vi "GDSLvIcon_GenerateIconText.vi"(1 "Text":T2, 2 "TextPixelHeight(5-30)":i32=7, 3 "Foreground color":u32(colorbox), 4 "Background color":u32(colorbox)=16777215, 5 "error in (no error)":errorcluster, 6 "Offset":cluster{"X":i32, "Y":i32}, 7 "Text Pixel width(32-FrameThicknes*2))":i32=30) -> (14 "X-Limited":bool, 15 "Y-Limited":bool, 17 "TextOut":u8[][](array[numeric]), 18 "TextBounds":T1, 19 "error out":errorcluster)   [LabVIEW 2020]
doc: "Applies a text in the template picture."
uses:
  <resource>/Framework/Providers/Open_GDS/ClassProviders/Common/LvIcon_class/subvis/GDSLvIcon_TextDataType.ctl
  <resource>/Framework/Providers/Open_GDS/ClassProviders/Common/LvIcon_class/GDSLvIcon_WordCompressionType.ctl
  <resource>/Framework/Providers/Open_GDS/ClassProviders/Common/LvIcon_class/GDSLvIcon_TextAlignment.ctl
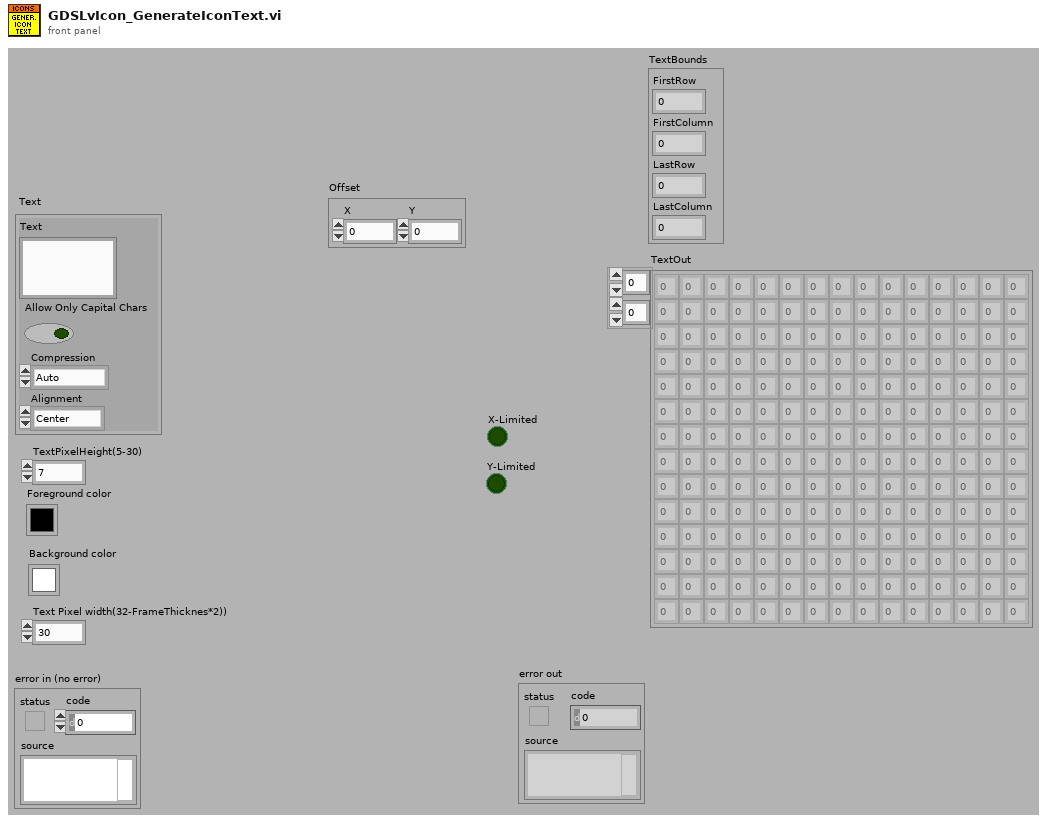
[diagram p1: front panel]
types:
  T1 = cluster{"FirstRow":i32, "FirstColumn":i32, "LastRow":i32, "LastColumn":i32}
  T2 = typedef "GDSLvIcon_TextDataType.ctl" = cluster{"Text":string, "Allow Only Capital Chars":bool, "Compression":T3, "Alignment":T4}
  T3 = typedef "GDSLvIcon_WordCompressionType.ctl" = enum16{"Auto", "On", "Off"}
  T4 = typedef "GDSLvIcon_TextAlignment.ctl" = enum16{"Center", "Left", "Right"}
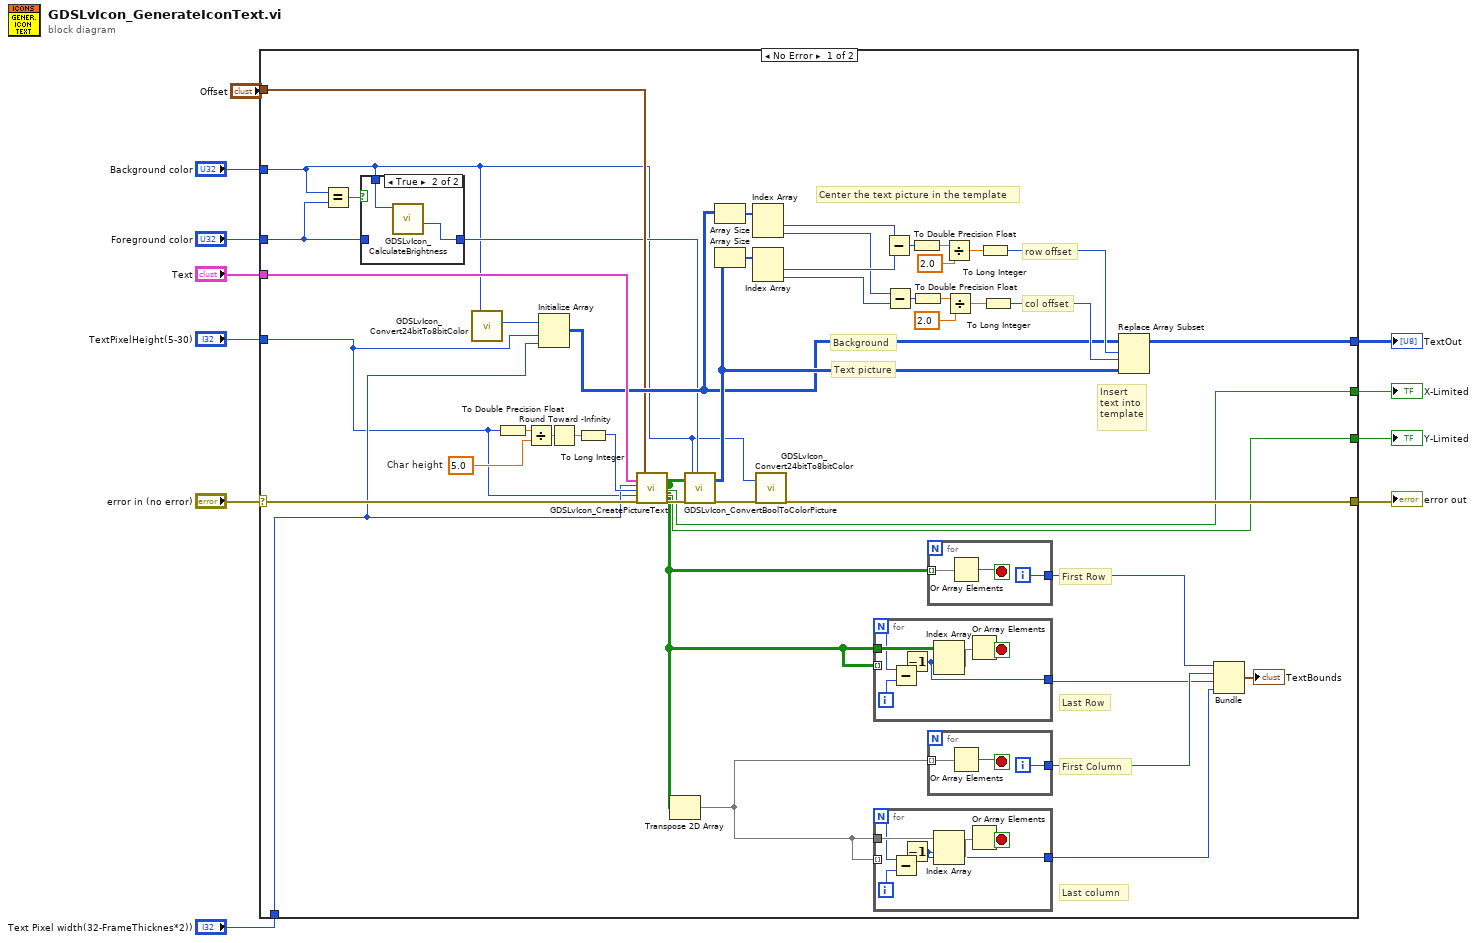
[diagram p0: block diagram]
diagram:
  n1 = case shown="No Error" "error in (no error)" {
    selector: "error in (no error)" -> [w34 w81]
    tunnel: [w36 w81] -> w10
    tunnel: "Foreground color" -> [w14 _]
    tunnel: "Background color" -> [w12 _]
    tunnel: "Text" -> [w57 _]
    tunnel: "TextPixelHeight(5-30)" -> [w26 _]
    tunnel: [w27 _] -> w5
    tunnel: "Text Pixel width(32-FrameThicknes*2))" -> [w29 _]
    tunnel: "Offset" -> [w25 _]
    tunnel: [w24 _] -> w2
    tunnel: [w23 _] -> w1
    frame No Error {
      w56 = 5.0  # Char height
      # "Last column"
      # "First Column"
      # "Last Row"
      # "First Row"
      # "Insert\ntext into\ntemplate"
      # "col offset"
      # "row offset"
      # "Center the text picture in the template"
      # "Text picture"
      # "Background"
      n2 = Equal?(x=w12, y=w14) -> (x = y?=w15:bool)
      n3 = case shown="True" w15 {
        tunnel: w14 -> [w58 _]
        tunnel: [w58 w59] -> w13
        tunnel: w12 -> [_ w60]
        frame False {
        }
        frame True {
          n4 = call <resource>:"GDSLvIcon_CalculateBrightness.vi"("RGB Color In"=w60) -> ("SuggestedTextColor"=w59:u32)  [unwired: 8 in, 2 out]
        }
      }
      n5 = call <resource>:"GDSLvIcon_Convert24bitTo8bitColor.vi"("Color 24bit In"=w12) -> ("Color out(256)"=w35:u8)  [unwired: 15 in, 3 out]
      n6 = To Double Precision Float(number=w26) -> (double precision float=w55:dbl)
      n7 = Divide(x=w55, y=w56) -> (x/y=w54:dbl)
      n8 = Initialize Array(w35, w26, w29) -> (w28:u8[][])
      n9 = Round Toward -Infinity(1:w54) -> (0:w53:dbl)
      n10 = To Long Integer(number=w53) -> (32bit integer=w52:i32)
      n11 = call <resource>:"GDSLvIcon_CreatePictureText.vi"("Text"=w57, "Pixel width"=w29, "Max nr of rows"=w52, "Pixel height"=w26, "error in (no error)"=w34, "Offset"=w25) -> ("CharPicture"=w19:bool[][], "X-Limited"=w24:bool, "Y-Limited"=w23:bool, "error out"=w38:errorcluster)  [unwired: 10 in]
      n12 = Transpose 2D Array(2D array=w19) -> (transposed array=w18:bool[][])
      n13 = call <resource>:"GDSLvIcon_ConvertBoolToColorPicture.vi"("CharPicture"=w19, "error in (no error)"=w38, "Background color"=w12, "Foreground color"=w13) -> ("CharPicture out"=w30:u8[][], "error out"=w37:errorcluster)  [unwired: 14 in]
      n14 = Array Size(array=w28) -> (size(s)=w33:i32[])
      n15 = Array Size(array=w30) -> (size(s)=w51:i32[])
      n16 = Index Array(array=w33) -> (element #1=w32:i32, element #2=w31:i32)  [unwired: 2 in]
      n17 = Index Array(array=w51) -> (element #1=w50:i32, element #2=w43:i32)  [unwired: 2 in]
      n18 = call <resource>:"GDSLvIcon_Convert24bitTo8bitColor.vi"("Color 24bit In"=w12, "error in (no error)"=w37) -> ("error out"=w36:errorcluster)  [unwired: 14 in, 3 out]
      n19 = for {
        N -> [w75]
        tunnel: w19 -> [w76]
        tunnel: [w71] -> w20
        tunnel: w19 -> [_] mode=indexing
        i -> [w74]
        stop <- w77 stop-if-true
        n20 = Subtract(x=w75, y=w74) -> (x-y=w73:i32)
        n21 = Decrement(x=w73) -> (x-1=w71:i32)
        n22 = Index Array(array=w76, index (row)=w71) -> (element=w72:bool[])  [unwired: 1 in]
        n23 = Or Array Elements(Boolean array=w72) -> (logical OR=w77:bool)
      }
      n24 = for {
        N -> [w65]
        tunnel: w18 -> [w66]
        tunnel: w18 -> [_] mode=indexing
        tunnel: [w61] -> w17
        i -> [w64]
        stop <- w67 stop-if-true
        n25 = Subtract(x=w65, y=w64) -> (x-y=w63:i32)
        n26 = Decrement(x=w63) -> (x-1=w61:i32)
        n27 = Index Array(array=w66, index (row)=w61) -> (element=w62:bool[])  [unwired: 1 in]
        n28 = Or Array Elements(Boolean array=w62) -> (logical OR=w67:bool)
      }
      n29 = Subtract(x=w32, y=w50) -> (x-y=w49:i32)
      n30 = Subtract(x=w31, y=w43) -> (x-y=w44:i32)
      n31 = To Double Precision Float(number=w49) -> (double precision float=w47:dbl)
      n32 = To Double Precision Float(number=w44) -> (double precision float=w46:dbl)
      n33 = for {
        tunnel: w19 -> [w80] mode=indexing
        tunnel: [w78] -> w22
        i -> [w78]
        stop <- w79 stop-if-true
        n34 = Or Array Elements(Boolean array=w80) -> (logical OR=w79:bool)
      }
      n35 = for {
        tunnel: w18 -> [w70] mode=indexing
        tunnel: [w68] -> w21
        i -> [w68]
        stop <- w69 stop-if-true
        n36 = Or Array Elements(Boolean array=w70) -> (logical OR=w69:bool)
      }
      n37 = Divide(x=w47, y=2.0) -> (x/y=w42:dbl)
      n38 = Divide(x=w46, y=2.0) -> (x/y=w41:dbl)
      n39 = To Long Integer(number=w42) -> (32bit integer=w40:i32)
      n40 = To Long Integer(number=w41) -> (32bit integer=w39:i32)
      n41 = Replace Array Subset(array=w28, new element=w30, index (row)=w40, index (col)=w39) -> (w27:u8[][])
      n42 = Bundle(w22, w21, w20, w17) -> (→"TextBounds":cluster{i32, i32, i32, i32})  [unwired: 1 in]
    }
    frame Error {
    }
  }
  "error out" <- w10
  "TextOut" <- w5
  "Y-Limited" <- w1
  "X-Limited" <- w2
